vi "Create_Data_For_WS2813.vi"(11 "Color Box":u32(colorbox)) -> (3 "string":string)   [LabVIEW 2020, in "CTI-Scratchpad.lvlib"]
uses:
  CTI-Scratchpad.lvlib
panel:
  out "size(s)":i32
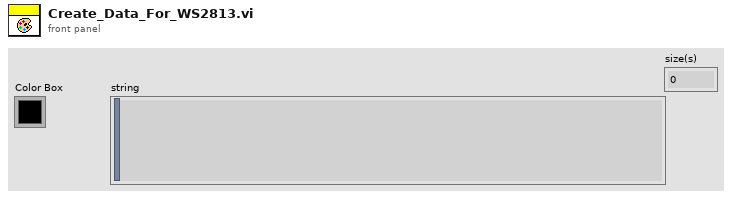
[diagram p1: front panel]
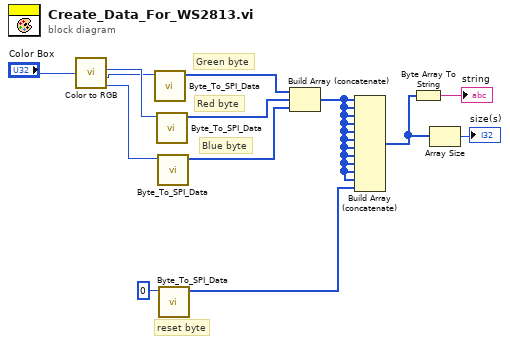
[diagram p0: block diagram]
diagram:
  # "reset byte"
  # "Blue byte"
  # "Red byte"
  # "Green byte"
  n1 = call <vilib>:"Color to RGB.vi"("Color"="Color Box") -> ("R"=w7:u8, "G"=w6:u8, "B"=w10:u8)  [unwired: 1 out]
  n2 = call "Byte_To_SPI_Data.vi"("Byte value"=w6) -> ("SPI Data"=w13:u8[])  [unwired: 10 in]
  n3 = call "Byte_To_SPI_Data.vi"("Byte value"=w7) -> ("SPI Data"=w9:u8[])  [unwired: 10 in]
  n4 = call "Byte_To_SPI_Data.vi"("Byte value"=w10) -> ("SPI Data"=w8:u8[])  [unwired: 10 in]
  n5 = call "Byte_To_SPI_Data.vi"("Byte value"=u8 0) -> ("SPI Data"=w2:u8[])  [unwired: 10 in]
  n6 = Build Array (concatenate)(w13, w9, w8) -> (w1:u8[])
  n7 = Build Array (concatenate)(w1, w1, w1, w1, w1, w1, w1, w1, w1, w1, w1, w2) -> (w4:u8[])
  n8 = Byte Array To String(unsigned byte array=w4) -> (string=→"string":string)
  n9 = Array Size(array=w4) -> (size(s)=→"size(s)":i32)
